vi "Read States.vi"(8 "error in (no error)":errorcluster, 11 "CSM-Helper in":refnum<class "CSM-Helper.lvclass">) -> (0 "error out":errorcluster, 2 "Value":string[](array[string]), 3 "CSM-Helper out":refnum<class "CSM-Helper.lvclass">)   [LabVIEW 2017, in "CSM-Helper.lvclass"]
doc: "### Read States.vi\n\n-- <b>Controls</b> --\n- <b>CSM-Helper in</b>: CSMHelper input\n\n-- <b>Indicators</b> --\n- <b>Value</b>:\n- <b>CSM-Helper out</b>: CSMHelper output"
uses:
  CSM-Helper.lvclass
  CSM-Helper.lvclass/CSM-Helper.ctl
  _Shared/CSM Shared.lvlib
  Communicable State Machine.lvlib
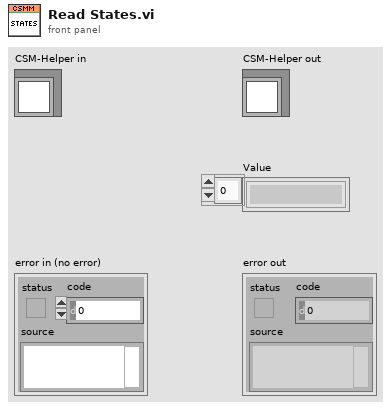
[diagram p1: front panel]
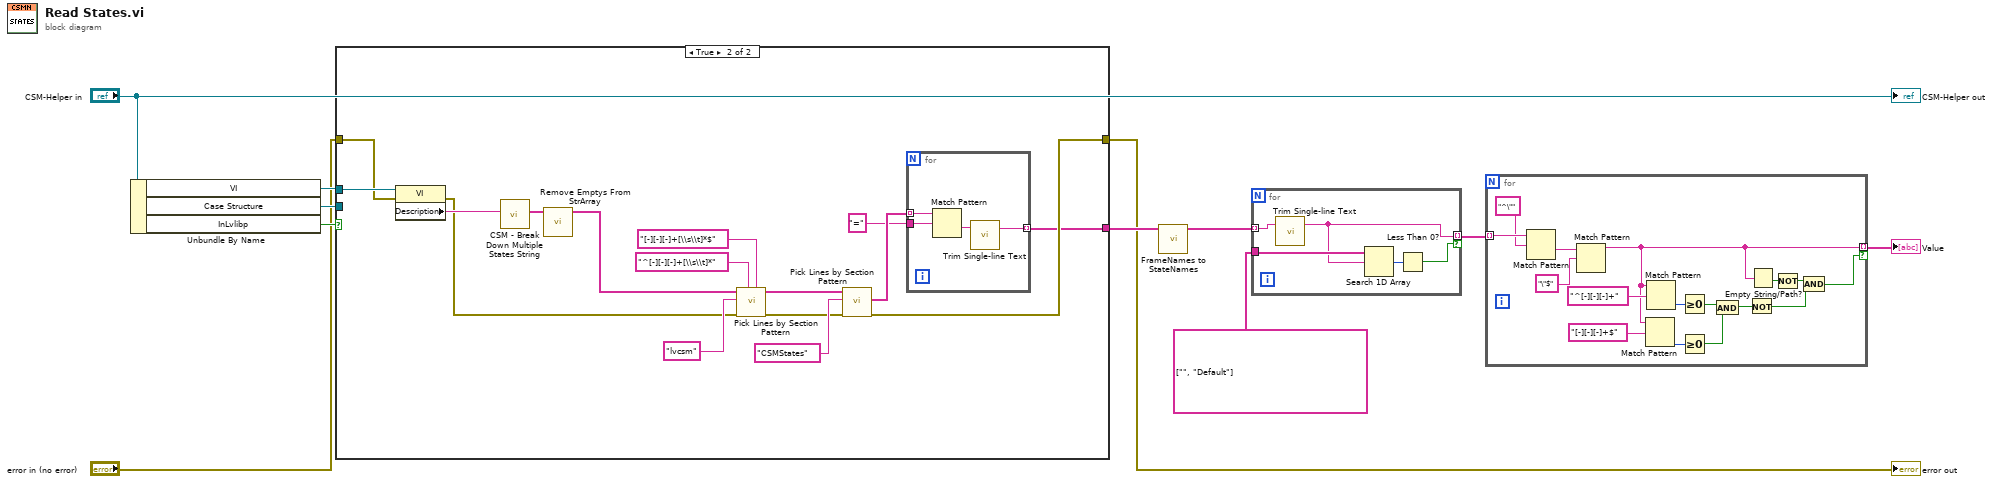
[diagram p0: block diagram]
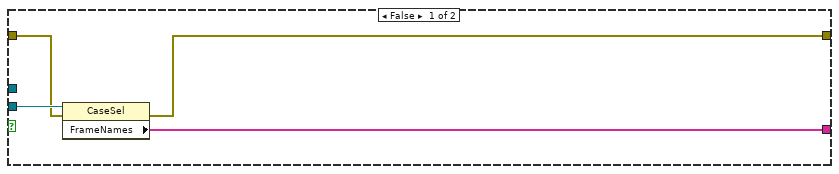
[diagram p2: hidden frame]
diagram:
  n1 = Unbundle By Name("CSM-Helper in") -> ("VI"=w4:refnum<vi>, "Case Structure"=w6:refnum<vi>, "InLvlibp"=w5:bool)
  n2 = case shown="True" w5 {
    tunnel: w6 -> [w15 _]
    tunnel: [w12 w25] -> w2
    tunnel: [w13 w28] -> w1
    tunnel: "error in (no error)" -> [w14 w29]
    tunnel: w4 -> [_ w30]
    frame False {
      n3 = property on="Property Node" class="CaseSel"(reference=w15, error in=w14) -> (error out=w13:errorcluster, "FrameNames"=w12:string[])  [unwired: 1 out]
    }
    frame True {
      n4 = property class="VI"(reference=w30, error in=w29) -> (error out=w22:errorcluster, "Description"=w23:string)  [unwired: 1 out]
      n5 = call "CSM - Break Down Multiple States String.vi"("States"=w23) -> ("Multiple States"=w17:string[])  [unwired: 10 in]
      n6 = call "Remove Emptys From StrArray.vi"("Array In"=w17) -> ("Array Out"=w16:string[])  [unwired: 10 in]
      n7 = call "Pick Lines by Section Pattern.vi"("RegExp Right(\"^[\")"="[-][-][-]+[\\s\\t]*$" ("RegExp Lef(\"^[\")"), "RegExp Lef(\"^[\")"="^[-][-][-]+[\\s\\t]*" ("RegExp Lef(\"^[\")"), "error in (no error)"=w22, "Session Name"="lvcsm" ("[] Session Name"), "Config Text List"=w16) -> ("error out"=w21:errorcluster, "Config Text List out"=w20:string[])  [unwired: 2 in, 3 out]
      n8 = call "Pick Lines by Section Pattern.vi"("error in (no error)"=w21, "Session Name"="CSMStates" ("[] Session Name"), "Config Text List"=w20) -> ("error out"=w28:errorcluster, "Session"=w27:string[])  [unwired: 4 in, 3 out]
      n9 = for {
        tunnel: w27 -> [w35] mode=indexing
        tunnel: "=" ("regular expression") -> [w34]
        tunnel: [w32] -> w25 mode=indexing
        n10 = Match Pattern(string=w35, regular expression=w34) -> (after substring=w33:string)  [unwired: 1 in, 3 out]
        n11 = call "Trim Single-line Text.vi"("single-line text"=w33) -> ("trimed text"=w32:string)  [unwired: 2 in]
      }
    }
  }
  "error out" <- w1
  n12 = call "FrameNames to StateNames.vi"("FrameNames"=w2) -> ("Array of Strings"=w7:string[])  [unwired: 10 in]
  n13 = for {
    tunnel: w7 -> [w40] mode=indexing
    tunnel: [w38] -> w11 mode=indexing if=w36
    tunnel: string[] ["", "Default"] ("items to filter") -> [w39]
    n14 = call "Trim Single-line Text.vi"("single-line text"=w40) -> ("trimed text"=w38:string)  [unwired: 2 in]
    n15 = Search 1D Array(1D array=w39, element=w38) -> (index of element=w37:i32)  [unwired: 1 in]
    n16 = Less Than 0?(x=w37) -> (x < 0?=w36:bool)
  }
  n17 = for {
    tunnel: w11 -> [w56] mode=indexing
    tunnel: [w41] -> w9 mode=indexing if=w45
    n18 = Match Pattern(string=w56, regular expression="^\"") -> (after substring=w54:string)  [unwired: 1 in, 3 out]
    n19 = Match Pattern(string=w54, regular expression="\"$") -> (before substring=w41:string)  [unwired: 1 in, 3 out]
    n20 = Match Pattern(string=w41, regular expression="[-][-][-]+$") -> (offset past match=w49:i32)  [unwired: 1 in, 3 out]
    n21 = Match Pattern(string=w41, regular expression="^[-][-][-]+") -> (offset past match=w50:i32)  [unwired: 1 in, 3 out]
    n22 = Greater Or Equal To 0?(x=w50) -> (x >= 0?=w48:bool)
    n23 = Greater Or Equal To 0?(x=w49) -> (x >= 0?=w47:bool)
    n24 = And(x=w48, y=w47) -> (x .and. y?=w46:bool)
    n25 = Not(x=w46) -> (.not. x?=w44:bool)
    n26 = Empty String/Path?(string/path=w41) -> (empty?=w43:bool)
    n27 = Not(x=w43) -> (.not. x?=w42:bool)
    n28 = And(x=w42, y=w44) -> (x .and. y?=w45:bool)
  }
  "Value" <- w9
  "CSM-Helper out" <- "CSM-Helper in"
